vi "Create Enum Accessor.vi"(8 "error in (no error)":errorcluster, 10 "message name":string, 11 "library in":refnum<vi>) -> (0 "error out":errorcluster, 3 "library out":refnum<vi>)   [LabVIEW 2019, in "gRPC Template Creation Utility.lvlib"]
uses:
  gRPC Template Creation Utility.lvlib
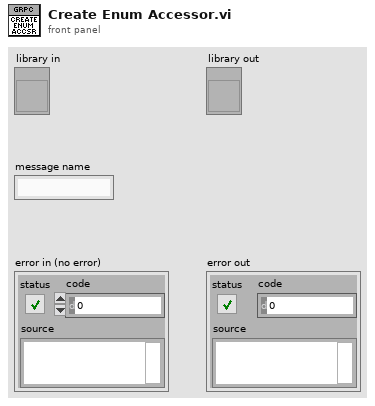
[diagram p1: front panel]
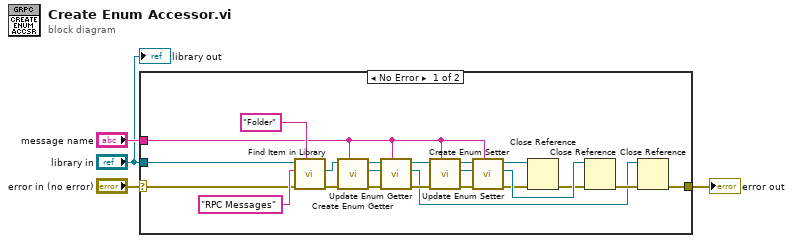
[diagram p0: block diagram]
diagram:
  n1 = case shown="No Error" "error in (no error)" {
    selector: "error in (no error)" -> [w23 w27]
    tunnel: "library in" -> [w22 _]
    tunnel: "message name" -> [w13 _]
    tunnel: [w24 w27] -> w4
    frame No Error {
      n2 = call "Find Item in Library.vi"("Item Type"="Folder", "error in (no error)"=w23, "Item Name"="RPC Messages", "Library item in"=w22) -> ("error out"=w20:errorcluster, "Project Item (Library Item)"=w21:refnum<vi>)  [unwired: 4 in, 2 out]
      n3 = call "Create Enum Getter.vi"("RPC Message Name"=w13, "error in (no error)"=w20, "RPC Messages Folder (ProjectItem) in"=w21) -> ("error out"=w17:errorcluster, "Message Getter out"=w18:refnum<vi>, "RPC Messages Folder (ProjectItem) out"=w19:refnum<vi>)  [unwired: 6 in]
      n4 = call "Update Enum Getter.vi"("RPC Message Name"=w13, "error in (no error)"=w17, "Message Getter in"=w18, "RPC Messages Folder (ProjectItem) in"=w19) -> ("error out"=w11:errorcluster, "Message Getter out"=w5:refnum<vi>, "RPC Messages Folder (ProjectItem) out"=w10:refnum<vi>)  [unwired: 5 in]
      n5 = call "Create Enum Setter.vi"("RPC Message Name"=w13, "error in (no error)"=w11, "RPC Messages Folder (ProjectItem) in"=w10) -> ("error out"=w14:errorcluster, "Message Setter out"=w15:refnum<vi>, "RPC Messages Folder (ProjectItem) out"=w16:refnum<vi>)  [unwired: 6 in]
      n6 = call "Update Enum Setter.vi"("RPC Message Name"=w13, "error in (no error)"=w14, "Message Getter in"=w15, "RPC Messages Folder (ProjectItem) in"=w16) -> ("error out"=w9:errorcluster, "Message Getter out"=w12:refnum<vi>, "RPC Messages Folder (ProjectItem) out"=w6:refnum<vi>)  [unwired: 5 in]
      n7 = Close Reference(reference=w6, error in (no error)=w9) -> (error out=w7:errorcluster)
      n8 = Close Reference(reference=w12, error in (no error)=w7) -> (error out=w8:errorcluster)
      n9 = Close Reference(reference=w5, error in (no error)=w8) -> (error out=w24:errorcluster)
    }
    frame Error {
    }
  }
  "error out" <- w4
  "library out" <- "library in"
